vi "Dequeue Frame.vi"(8 "error in":errorcluster, 11 "GUID":string) -> (0 "error out":errorcluster, 3 "Data":string[][](array[string]))   [LabVIEW 2025, in "CAN-LIN Raw Bus Capture.lvclass"]
uses:
  CAN-LIN Raw Bus Capture.lvclass
  CAN-LIN Raw Bus Capture.lvclass/CAN-LIN Raw Bus Capture.ctl
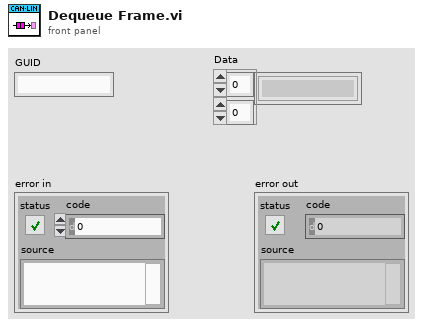
[diagram p1: front panel]
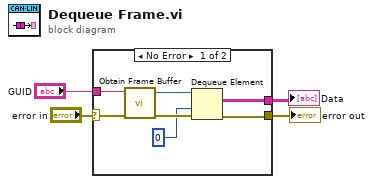
[diagram p0: block diagram]
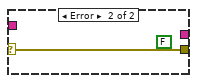
[diagram p2: hidden frame]
diagram:
  n1 = case shown="No Error" "error in" {
    selector: "error in" -> [w11 w12]
    tunnel: [w7 w12] -> w3
    tunnel: [w6 _] -> w2
    tunnel: "GUID" -> [w5 _]
    frame No Error {
      n2 = call "Obtain Frame Buffer.vi"("error in"=w11, "GUID"=w5) -> ("error out"=w10:errorcluster, "queue out"=w9:refnum<queue>)  [unwired: 8 in]
      n3 = Dequeue Element(queue=w9, timeout in ms (-1)=0, error in (no error)=w10) -> (element=w6:string[][], error out=w7:errorcluster)  [unwired: 2 out]
    }
    frame Error {
      (unwired) FALSE ("overflow?")
    }
  }
  "error out" <- w3
  "Data" <- w2
